vi "Example I2C ADXL345.vi"() -> ()   [LabVIEW 2025]
uses:
  <vilib>/platform/TimedLoop/XDataNode/XDataNode.xnode
  <vilib>/Platform/TimedLoop/XDataNode/nitl_modes.ctl
  <vilib>/Platform/TimedLoop/XDataNode/XDNodeRunTimeDep.lvlib
  <vilib>/Platform/TimedLoop/XDataNode/wakeup.ctl
  <vilib>/Platform/TimedLoop/XDataNode/timing_clust.ctl
  wiringPi.lvlib
  I2C/Internal/I2C Write Reg 8.vi
  I2C/Internal/I2C Read Reg Block.vi
panel:
  out "Aceleration":cluster{dbl, dbl, dbl}(graph)
  in  "stop":bool
  in  "I2C Slave Address (0x1D o 0x53)":u8=83 format="%.0x"
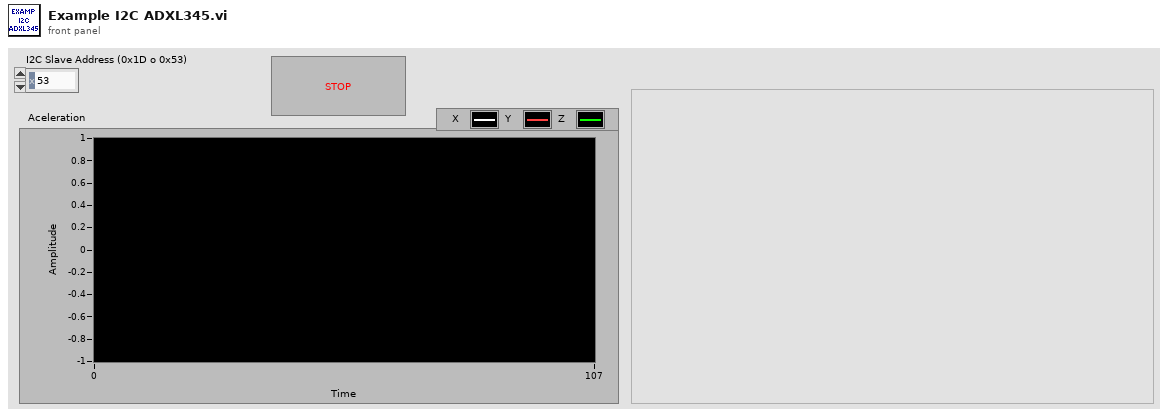
[diagram p1: front panel]
types:
  T1 = enum8{"DEVID", "-1-", "-2-", "-3-", "-4-", "-5-", "-6-", "-7-", "-8-", "-9-", "-A-", "-B-", "-C-", "-D-", "-E-", "-F-", "-10-", "-11-", "-12-", "-13-", "-14-", "-15-", "-16", "-17", "-18-", "-19-", "-1A-", "-1B-", "-1C-", "THRESH_TAP", "OFSX", "OFSY", "OFSZ", "DUR", "Latent", "Window", "THRESH_ACT", "THRESH_INACT", "TIME_INACT", "ACT_INACT_CTL", "THRESH_FF", "TIME_FF", "TAP_AXES", "ACT_TAP_STATUS", "BW_RATE", "POWER_CTL", "INT_ENABLE", "INT_MAP", "INT_SOURCE", "DATA_FORMAT", "DATAX0", "DATAX1", "DATAY0", "DATAY1", "DATAZ0", "DATAZ1", "FIFO_CTL", "FIFO_STATUS"}
  T2 = typedef "wiringPi.lvlib/I2C Device.ctl" = i32
  T3 = typedef "XDNodeRunTimeDep.lvlib/timing_clust.ctl" = cluster{"Expected End [f-1]":u64, "Actual End [f-1]":u64, "Finished Late? [f-1]":bool, "Expected End [i-1]":u64, "Actual End [i-1]":u64, "Finished Late? [i-1]":bool, "Expected Start [i]":u64, "Actual Start [i]":u64, "Expected Start [f]":u64, "Actual Start [f]":u64, "Source Name":string, "Structure Name":string, "Period":i64, "Deadline":i64, "Offset":i64, "Start":i64, "Priority":i32, "Timeout":i32, "Mode":T4, "Wakeup Reason":T5, "Error":errorcluster, "Source Type":string, "Secondary Source Type":string, "Global End Time":u64, "Global Start Time":u64, "Frame Duration":u64, "Iteration Duration":u64, "Assigned CPU":i32, "I/O Scan Engine Mode":u32}
  T4 = typedef "XDNodeRunTimeDep.lvlib/nitl_modes.ctl" = enum32{"No Change", "Process missed periods, maintain original phase", "Discard missed periods, maintain original phase", "Process missed periods, ignore original phase", "Discard missed periods, ignore original phase"}
  T5 = typedef "XDNodeRunTimeDep.lvlib/wakeup.ctl" = enum32{"Normal", "Aborted", "Asynchronous wakeup", "Timing source error", "Timed loop error", "Timeout"}
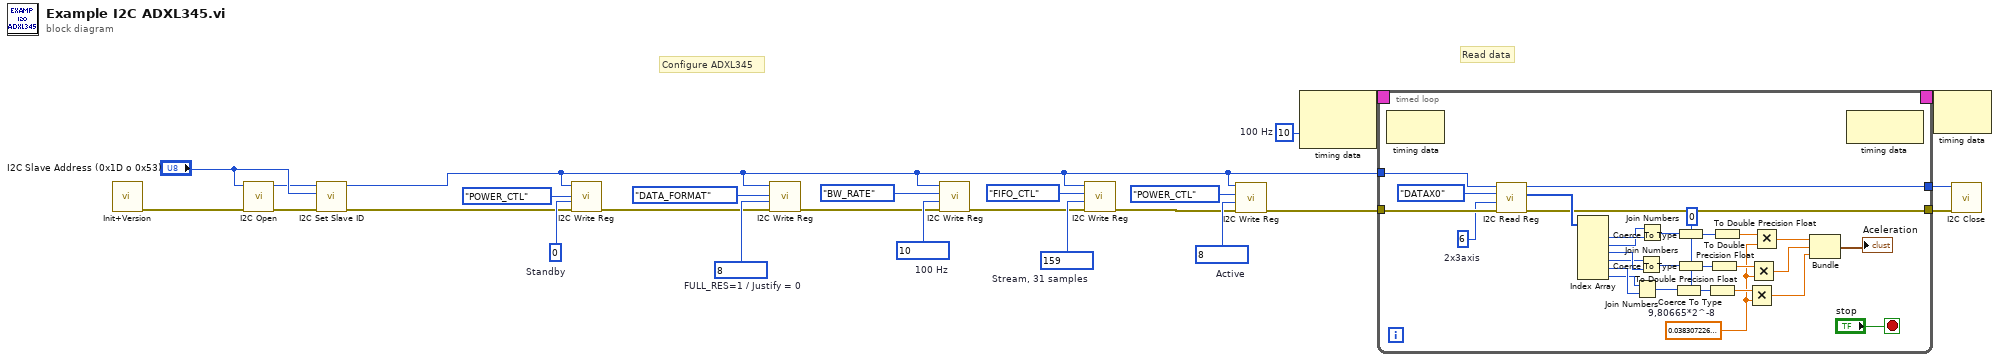
[diagram p0: block diagram]
diagram:
  w9 = i64 10  # 100 Hz
  w17 = u8 10  # 100 Hz
  w21 = u8 159  # Stream, 31 samples
  w23 = u8 8  # FULL_RES=1 / Justify = 0
  w18 = u8 8  # Active
  w26 = u8 0  # Standby
  # "Read data"
  # "Configure ADXL345"
  n1 = call "Init+Version.vi"() -> ("error out"=w1:errorcluster)  [unwired: 8 in, 3 out]
  n2 = call "I2C Open.vi"("error in (no error)"=w1, "Slave Id"="I2C Slave Address (0x1D o 0x53)") -> ("error out"=w3:errorcluster, "I2C Device out"=w4:T2)  [unwired: 8 in]
  n3 = call "I2C Set Slave ID.vi"("error in (no error)"=w3, "Slave Id"="I2C Slave Address (0x1D o 0x53)", "I2C Device"=w4) -> ("error out"=w2:errorcluster, "I2C Device out"=w6:T2)  [unwired: 7 in]
  n4 = call-poly "I2C Write Reg.vi"("error in (no error)"=w2, "Value"=w26, "Register"=T1."POWER_CTL" ("Dirección"), "I2C Device"=w6) -> ("error out"=w12:errorcluster)  [unwired: 6 in, 1 out]
  n5 = call-poly "I2C Write Reg.vi"("error in (no error)"=w12, "Value"=w23, "Register"=T1."DATA_FORMAT" ("Dirección"), "I2C Device"=w6) -> ("error out"=w16:errorcluster)  [unwired: 6 in, 1 out]
  n6 = call-poly "I2C Write Reg.vi"("error in (no error)"=w16, "Value"=w17, "Register"=T1."BW_RATE" ("Dirección"), "I2C Device"=w6) -> ("error out"=w14:errorcluster)  [unwired: 6 in, 1 out]
  n7 = call-poly "I2C Write Reg.vi"("error in (no error)"=w14, "Value"=w21, "Register"=T1."FIFO_CTL" ("Dirección"), "I2C Device"=w6) -> ("error out"=w15:errorcluster)  [unwired: 6 in, 1 out]
  n8 = call-poly "I2C Write Reg.vi"("error in (no error)"=w15, "Value"=w18, "Register"=T1."POWER_CTL" ("Dirección"), "I2C Device"=w6) -> ("error out"=w13:errorcluster)  [unwired: 6 in, 1 out]
  n9 = node-c288(w9) -> (w11:T3)  [unwired: 1 in]
  n10 = timed-loop {
    timing: w11 -> [_]
    timing-out: [_] -> w10
    tunnel: w13 -> [w55]
    tunnel: w6 -> [w53]
    tunnel: [w32] -> w7
    tunnel: [w31] -> w8
    stop <- "stop" stop-if-true
    w38 = i16 0 ("number")
    w35 = 0.0383072265625  # 9,80665*2^-8
    w34 = u32 6  # 2x3axis
    n11 = node-c288() -> ()  [unwired: 1 in, 1 out]
    n12 = call-poly "I2C Read Reg.vi"("error in (no error)"=w55, "Size"=w34, "Register"=T1."DATAX0" ("Address"), "I2C Device"=w53) -> ("error out"=w31:errorcluster, "Values"=w49:u8[], "I2C Device out"=w32:T2)  [unwired: 5 in]
    n13 = Index Array(array=w49) -> (element #1=w48:u8, element #2=w47:u8, element #3=w40:u8, element #4=w39:u8, element #5=w37:u8, element #6=w36:u8)  [unwired: 6 in]
    n14 = Join Numbers(hi=w36, lo=w37) -> ((hi.lo)=w42:u16)
    n15 = Join Numbers(hi=w39, lo=w40) -> ((hi.lo)=w41:u16)
    n16 = Join Numbers(hi=w47, lo=w48) -> ((hi.lo)=w50:u16)
    n17 = Coerce To Type(0:w42, 1:w38) -> (2:w43:i16)
    n18 = Coerce To Type(0:w50, 1:w38) -> (2:w51:i16)
    n19 = Coerce To Type(0:w41, 1:w38) -> (2:w46:i16)
    n20 = To Double Precision Float(number=w43) -> (double precision float=w44:dbl)
    n21 = To Double Precision Float(number=w46) -> (double precision float=w45:dbl)
    n22 = To Double Precision Float(number=w51) -> (double precision float=w52:dbl)
    n23 = Multiply(x=w44, y=w35) -> (x*y=w28:dbl)
    n24 = Multiply(x=w45, y=w35) -> (x*y=w29:dbl)
    n25 = Multiply(x=w52, y=w35) -> (x*y=w30:dbl)
    n26 = Bundle(w30, w29, w28) -> (→"Aceleration":cluster{dbl, dbl, dbl})  [unwired: 1 in]
    n27 = node-c288() -> ()  [unwired: 1 in, 1 out]
  }
  n28 = node-c288(w10) -> ()  [unwired: 1 out]
  n29 = call "I2C Close.vi"("error in (no error)"=w8, "I2C Device"=w7) -> ()  [unwired: 9 in, 1 out]
